vi "Built Copyrights Text.vi"(0 "Description in":string, 5 "Licence Text":string, 11 "error in":errorcluster) -> (4 "Description out":string, 15 "error out":errorcluster)   [LabVIEW 2016, in "SLL Add Copyright.lvlib"]
uses:
  SLL Add Copyright.lvlib
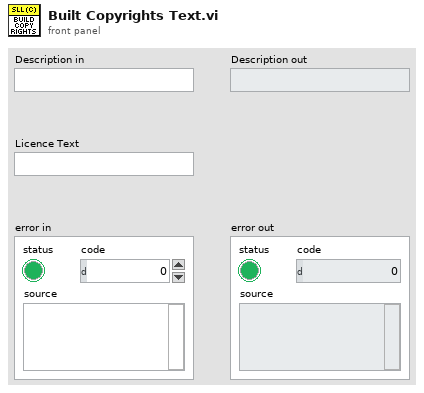
[diagram p1: front panel]
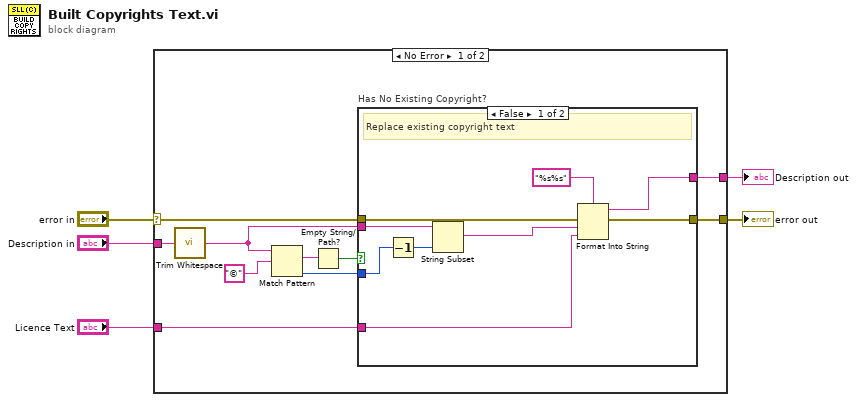
[diagram p0: block diagram]
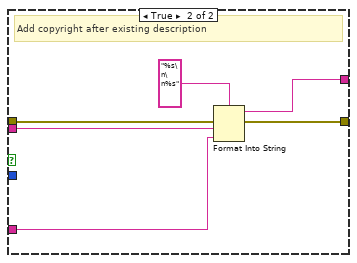
[diagram p2: hidden frame]
diagram:
  n1 = case shown="No Error" "error in" {
    selector: "error in" -> [w10 w32]
    tunnel: "Licence Text" -> [w11 _]
    tunnel: "Description in" -> [w9 w31]
    tunnel: [w8 w32] -> w2
    tunnel: [w7 w31] -> w1
    frame No Error {
      n2 = call <vilib>:"Trim Whitespace.vi"("string"=w9) -> ("trimmed string"=w6:string)  [unwired: 1 in]
      n3 = Match Pattern(string=w6, regular expression="©") -> (match substring=w14:string, offset past match=w12:i32)  [unwired: 1 in, 2 out]
      n4 = Empty String/Path?(string/path=w14) -> (empty?=w13:bool)
      n5 = case "Has No Existing Copyright?" shown="False" w13 {
        tunnel: [w23 w29] -> w8
        tunnel: w10 -> [w24 w30]
        tunnel: w6 -> [w20 w28]
        tunnel: [w21 w26] -> w7
        tunnel: w12 -> [w19 _]
        tunnel: w11 -> [w16 w25]
        frame False {
          # "Replace existing copyright text"
          n6 = Decrement(x=w19) -> (x-1=w17:i32)
          n7 = String Subset(string=w20, length (rest)=w17) -> (substring=w18:string)  [unwired: 1 in]
          n8 = Format Into String(format string="%s%s", error in=w24, w18, w16) -> (resulting string=w21:string, error out=w23:errorcluster)  [unwired: 1 in]
        }
        frame True {
          # "Add copyright after existing description"
          n9 = Format Into String(format string="%s\n\n%s", error in=w30, w28, w25) -> (resulting string=w26:string, error out=w29:errorcluster)  [unwired: 1 in]
        }
      }
    }
    frame Error {
    }
  }
  "error out" <- w2
  "Description out" <- w1
